vi "Test Data Dictionary API.vi"(8 "error in (no error)":errorcluster) -> (0 "error out":errorcluster)   [LabVIEW 2019]
uses:
  <vilib>/addons/_JKI Toolkits/Caraya/classes/Test/Test.lvclass
  LV-Data/LV-Data.lvclass
  LV-Data/Typedefs/Dictionary--cluster.ctl
  <vilib>/addons/_JKI Toolkits/Caraya/classes/Assert/Assert Equal Value and Type_Variant.vi
  <vilib>/addons/_JKI Toolkits/Caraya/classes/Assert/Assert.lvclass
  <vilib>/addons/_JKI Toolkits/Caraya/classes/Assert/Assert Not Error.vi
  <vilib>/numeric/Random Number (Range) I64.vi
  <vilib>/addons/_JKI Toolkits/Caraya/classes/Assert/Assert Error.vi
  LV-Data/API/XY-Data to Dictionary (Multiple).vi
  <vilib>/addons/_JKI Toolkits/Caraya/classes/Assert/Assert True.vi
  23d4e9fe-76af-4850-a45f-cc3c43636315.vi
  e87061af-0e9d-4de5-82b0-76289080f700.vi
  4053e775-25cb-4fab-9d61-351c3e686d1c.vi
  a8829717-a93e-4f97-b07c-db7713c6d1ae.vi
  8a392996-710f-4540-91e5-b205ccce4721.vi
  762a9f32-66e4-4e95-983a-dc45b51801a0.vi
  5820b508-eaf6-40a5-971f-30b0e9a2b10e.vi
  c95faebc-65c2-4475-abf8-9dea7ac9bcab.vi
  19599af3-a2bf-4e75-96ae-3692d4015444.vi
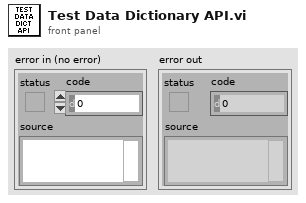
[diagram p1: front panel]
types:
  T1 = typedef "LV-Data.lvclass/Dictionary--cluster.ctl" = cluster{"key":string, "value":variant}
  T2 = typedef "LV-Data.lvclass/Map Variant--map.ctl" = map{string, variant}
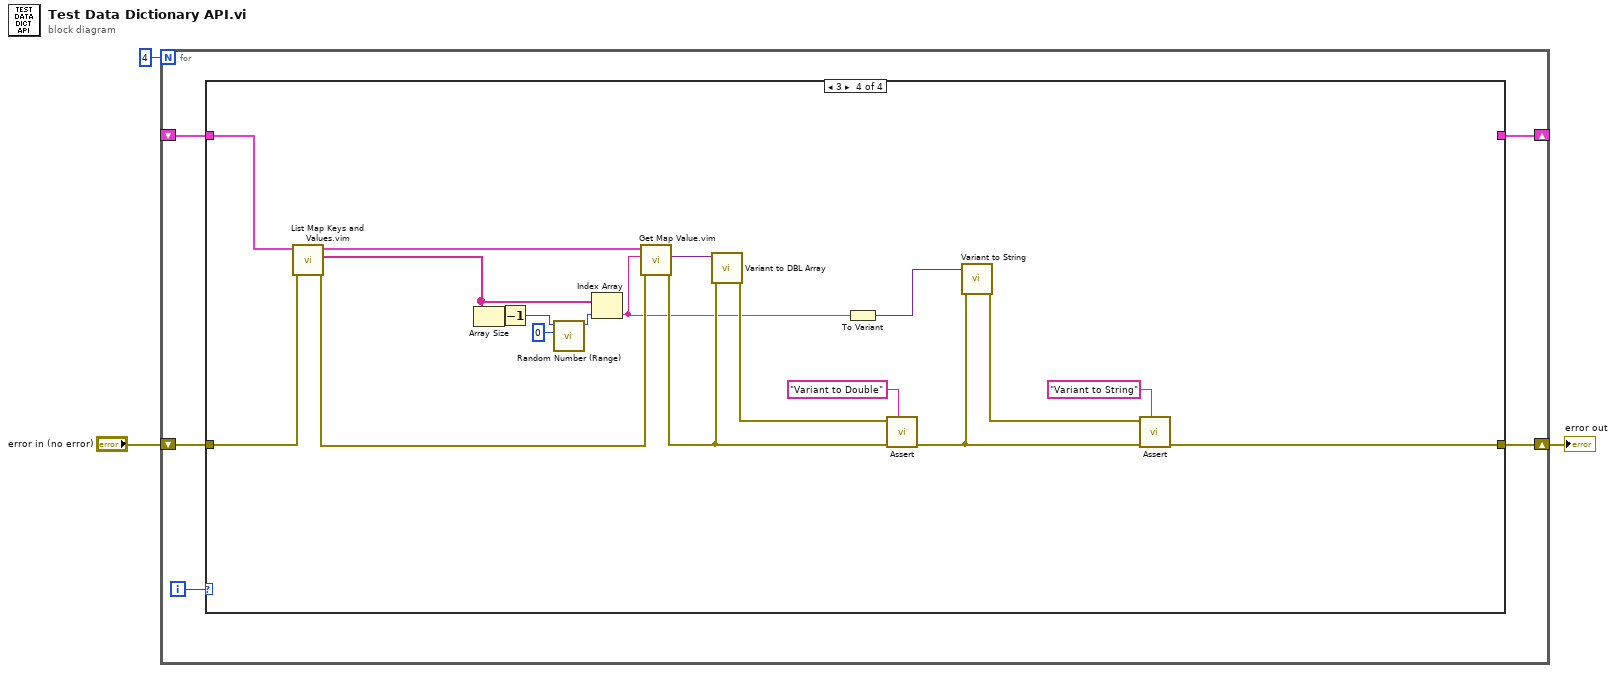
[diagram p0: block diagram]
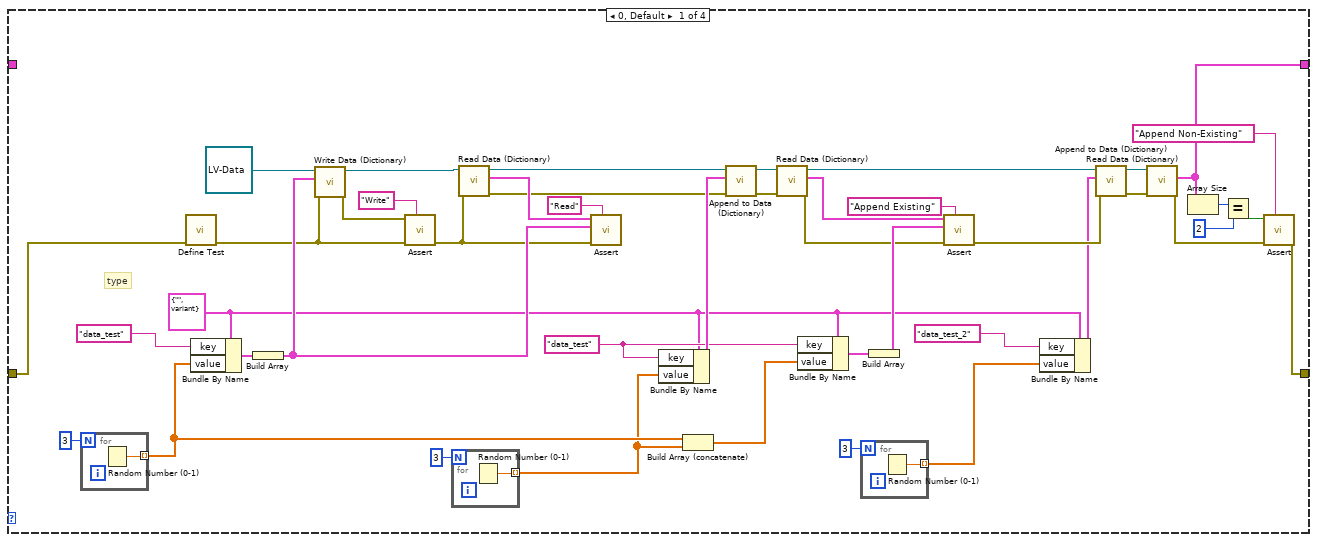
[diagram p2: hidden frame]
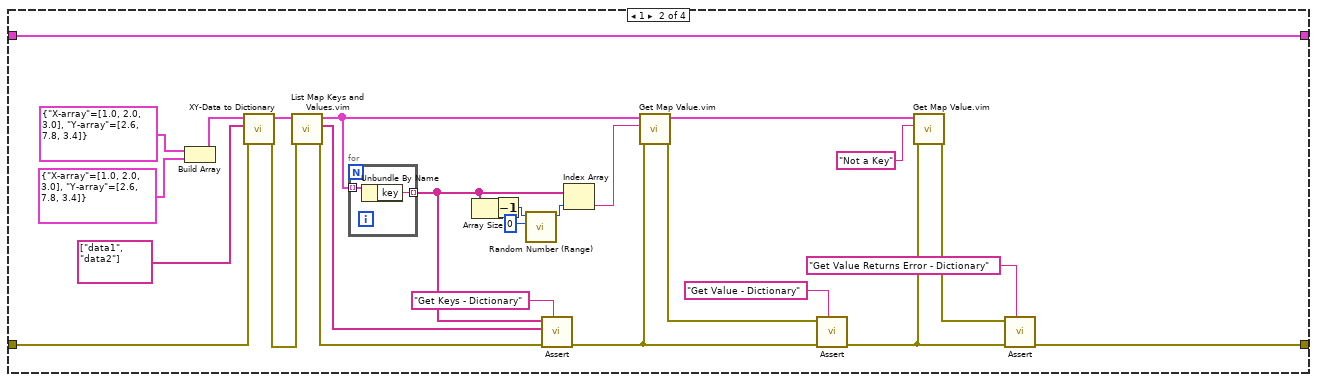
[diagram p3: hidden frame]
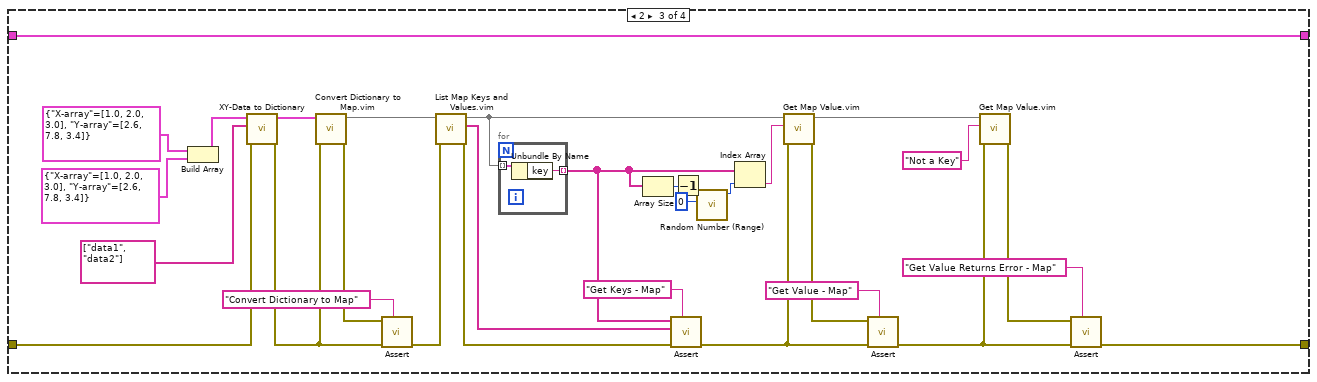
[diagram p4: hidden frame]
diagram:
  n1 = for {
    N: 4 -> [_]
    shift-right: [w7] -> w2
    shift-left: "error in (no error)" -> [w6]
    shift-right: [w5] -> _
    shift-left: _ -> [w4]
    i -> [w8]
    n2 = case shown="3" w8 {
      tunnel: [w17 w58 w87 w120] -> w7
      tunnel: w6 -> [w16 w60 w89 w130]
      tunnel: [w9 w56 w85 _] -> w5
      tunnel: w4 -> [_ w56 w85 w133]
      frame 0, Default {
        w43 = "data_test" ("key")
        w35 = T1 {"key"="", "value"=variant} ("key-value")
        # "type"
        n3 = for {
          N: 3 -> [_]
          tunnel: [w55] -> w14 mode=indexing
          n4 = Random Number (0-1)() -> (number: 0 to 1=w55:dbl)
        }
        n5 = call <vilib>:"Define Test.vi"("error in (no error)"=w16) -> ("error out"=w24:errorcluster)  [unwired: 10 in]
        n6 = Bundle By Name(cluster=w35, "key"="data_test", "value"=w14) -> (w51:T1)
        n7 = Build Array(w51) -> (w48:T1[])
        n8 = call "Write Data (Dictionary).vi"("error in (no error)"=w24, "Data (Dictionary)"=w48, "Data Save"=refnum<class "LV-Data.lvclass"> refnum) -> ("error out"=w25:errorcluster, "Data Save out"=w27:refnum<class "LV-Data.lvclass">)  [unwired: 7 in]
        n9 = call-poly <vilib>:"Assert.vi"("Label"="Write", "error in (no error)"=w24, "Not Error?"=w25) -> ("error out"=w26:errorcluster)  [unwired: 8 in]
        n10 = for {
          N: 3 -> [_]
          tunnel: [w54] -> w12 mode=indexing
          n11 = Random Number (0-1)() -> (number: 0 to 1=w54:dbl)
        }
        n12 = call "Read Data (Dictionary).vi"("error in (no error)"=w26, "Data Save"=w27) -> ("error out"=w23:errorcluster, "Data (Dictionary)"=w28:T1[], "Data Save out"=w22:refnum<class "LV-Data.lvclass">)  [unwired: 7 in]
        n13 = call-poly <vilib>:"Assert.vi"("Label"="Read", "error in (no error)"=w26, "Y"=w48, "X"=w28) -> ()  [unwired: 7 in, 1 out]
        n14 = Bundle By Name(cluster=w35, "key"=w43, "value"=w12) -> (w46:T1)
        n15 = Build Array (concatenate)(w14, w12) -> (w18:dbl[])
        n16 = call "Append to Data (Dictionary).vi"("error in (no error)"=w23, "key-value"=w46, "Data Save"=w22) -> ("error out"=w45:errorcluster, "Data Save out"=w44:refnum<class "LV-Data.lvclass">)  [unwired: 7 in]
        n17 = call "Read Data (Dictionary).vi"("error in (no error)"=w45, "Data Save"=w44) -> ("error out"=w21:errorcluster, "Data (Dictionary)"=w20:T1[], "Data Save out"=w19:refnum<class "LV-Data.lvclass">)  [unwired: 7 in]
        n18 = Bundle By Name(cluster=w35, "key"=w43, "value"=w18) -> (w42:T1)
        n19 = for {
          N: 3 -> [_]
          tunnel: [w53] -> w10 mode=indexing
          n20 = Random Number (0-1)() -> (number: 0 to 1=w53:dbl)
        }
        n21 = Build Array(w42) -> (w41:T1[])
        n22 = call-poly <vilib>:"Assert.vi"("Label"="Append Existing", "error in (no error)"=w21, "Y"=w41, "X"=w20) -> ("error out"=w37:errorcluster)  [unwired: 7 in]
        n23 = Bundle By Name(cluster=w35, "key"="data_test_2", "value"=w10) -> (w34:T1)
        n24 = call "Append to Data (Dictionary).vi"("error in (no error)"=w37, "key-value"=w34, "Data Save"=w19) -> ("error out"=w38:errorcluster, "Data Save out"=w39:refnum<class "LV-Data.lvclass">)  [unwired: 7 in]
        n25 = call "Read Data (Dictionary).vi"("error in (no error)"=w38, "Data Save"=w39) -> ("error out"=w30:errorcluster, "Data (Dictionary)"=w9:T1[])  [unwired: 7 in, 1 out]
        n26 = Array Size(array=w9) -> (size(s)=w33:i32)
        n27 = Equal?(x=w33, y=2) -> (x = y?=w31:bool)
        n28 = call-poly <vilib>:"Assert.vi"("Label"="Append Non-Existing", "error in (no error)"=w30, "True?"=w31) -> ("error out"=w17:errorcluster)  [unwired: 8 in]
      }
      frame 1 {
        n29 = Build Array(cluster{"X-array":dbl[], "Y-array":dbl[]} {"X-array"=[1.0, 2.0, 3.0], "Y-array"=[2.6, 7.8, 3.4]} ("XY-data in"), cluster{"X-array":dbl[], "Y-array":dbl[]} {"X-array"=[1.0, 2.0, 3.0], "Y-array"=[2.6, 7.8, 3.4]} ("XY-data in")) -> (w69:cluster{"X-array":dbl[], "Y-array":dbl[]}[])
        n30 = call-poly "XY-Data to Dictionary.vi"("error in (no error)"=w60, "Names"=string[] ["data1", "data2"], "XY-data in"=w69) -> ("error out"=w59:errorcluster, "Data (Dictionary)"=w70:T1[])  [unwired: 7 in]
        n31 = call "List Map Keys and Values.vim"("error in (no error)"=w59, "map in"=w70) -> ("error out"=w72:errorcluster, "Keys"=w71:string[], "map out"=w73:T1[])  [unwired: 6 in, 1 out]
        n32 = for {
          tunnel: w73 -> [w84] mode=indexing
          tunnel: [w83] -> w76 mode=indexing
          n33 = Unbundle By Name(w84) -> ("key"=w83:string)
        }
        n34 = Array Size(array=w76) -> (size(s)=w74:i32)
        n35 = Decrement(x=w74) -> (x-1=w57:i32)
        n36 = call-poly <vilib>:"Random Number (Range).vi"("lower bound (-100)"=i64 0, "upper bound (100)"=w57) -> ("number"=w75:i64)  [unwired: 9 in]
        n37 = call-poly <vilib>:"Assert.vi"("Label"="Get Keys - Dictionary", "error in (no error)"=w72, "Y"=w71, "X"=w76) -> ("error out"=w79:errorcluster)  [unwired: 7 in]
        n38 = Index Array(array=w76, index=w75) -> (element=w77:string)
        n39 = call "Get Map Value.vim"("error in (no error)"=w79, "Key"=w77, "map in"=w73) -> ("error out"=w78:errorcluster, "map out"=w80:T1[])  [unwired: 6 in, 1 out]
        n40 = call-poly <vilib>:"Assert.vi"("Label"="Get Value - Dictionary", "error in (no error)"=w79, "Not Error?"=w78) -> ("error out"=w82:errorcluster)  [unwired: 8 in]
        n41 = call "Get Map Value.vim"("error in (no error)"=w82, "Key"="Not a Key", "map in"=w80) -> ("error out"=w81:errorcluster)  [unwired: 6 in, 2 out]
        n42 = call-poly <vilib>:"Assert.vi"("Label"="Get Value Returns Error - Dictionary", "error in (no error)"=w82, "Error?"=w81) -> ("error out"=w58:errorcluster)  [unwired: 8 in]
      }
      frame 2 {
        n43 = Build Array(cluster{"X-array":dbl[], "Y-array":dbl[]} {"X-array"=[1.0, 2.0, 3.0], "Y-array"=[2.6, 7.8, 3.4]} ("XY-data in"), cluster{"X-array":dbl[], "Y-array":dbl[]} {"X-array"=[1.0, 2.0, 3.0], "Y-array"=[2.6, 7.8, 3.4]} ("XY-data in")) -> (w94:cluster{"X-array":dbl[], "Y-array":dbl[]}[])
        n44 = call-poly "XY-Data to Dictionary.vi"("error in (no error)"=w89, "Names"=string[] ["data1", "data2"], "XY-data in"=w94) -> ("error out"=w88:errorcluster, "Data (Dictionary)"=w90:T1[])  [unwired: 7 in]
        n45 = call "Convert Dictionary to Map.vim"("error in (no error)"=w88, "Data (Dictionary)"=w90) -> ("error out"=w101:errorcluster, "map out"=w104:T2)  [unwired: 8 in]
        n46 = call-poly <vilib>:"Assert.vi"("Label"="Convert Dictionary to Map", "error in (no error)"=w88, "Not Error?"=w101) -> ("error out"=w102:errorcluster)  [unwired: 8 in]
        n47 = call "List Map Keys and Values.vim"("error in (no error)"=w102, "map in"=w104) -> ("error out"=w103:errorcluster, "Keys"=w105:string[], "map out"=w109:T2)  [unwired: 6 in, 1 out]
        n48 = for {
          tunnel: w109 -> [w117] mode=indexing
          tunnel: [w116] -> w107 mode=indexing
          n49 = Unbundle By Name(w117) -> ("key"=w116:string)
        }
        n50 = Array Size(array=w107) -> (size(s)=w106:i32)
        n51 = call-poly <vilib>:"Assert.vi"("Label"="Get Keys - Map", "error in (no error)"=w103, "Y"=w105, "X"=w107) -> ("error out"=w112:errorcluster)  [unwired: 7 in]
        n52 = Decrement(x=w106) -> (x-1=w86:i32)
        n53 = call-poly <vilib>:"Random Number (Range).vi"("lower bound (-100)"=i64 0, "upper bound (100)"=w86) -> ("number"=w108:i64)  [unwired: 9 in]
        n54 = Index Array(array=w107, index=w108) -> (element=w110:string)
        n55 = call "Get Map Value.vim"("error in (no error)"=w112, "Key"=w110, "map in"=w109) -> ("error out"=w111:errorcluster, "map out"=w113:T2)  [unwired: 6 in, 1 out]
        n56 = call-poly <vilib>:"Assert.vi"("Label"="Get Value - Map", "error in (no error)"=w112, "Not Error?"=w111) -> ("error out"=w115:errorcluster)  [unwired: 8 in]
        n57 = call "Get Map Value.vim"("error in (no error)"=w115, "Key"="Not a Key", "map in"=w113) -> ("error out"=w114:errorcluster)  [unwired: 6 in, 2 out]
        n58 = call-poly <vilib>:"Assert.vi"("Label"="Get Value Returns Error - Map", "error in (no error)"=w115, "Error?"=w114) -> ("error out"=w87:errorcluster)  [unwired: 8 in]
      }
      frame 3 {
        n59 = call "List Map Keys and Values.vim"("error in (no error)"=w130, "map in"=w133) -> ("error out"=w129:errorcluster, "Keys"=w131:string[], "map out"=w132:T1[])  [unwired: 6 in, 1 out]
        n60 = Array Size(array=w131) -> (size(s)=w135:i32)
        n61 = Decrement(x=w135) -> (x-1=w124:i32)
        n62 = call-poly <vilib>:"Random Number (Range).vi"("lower bound (-100)"=i64 0, "upper bound (100)"=w124) -> ("number"=w136:i64)  [unwired: 9 in]
        n63 = Index Array(array=w131, index=w136) -> (element=w119:string)
        n64 = call "Get Map Value.vim"("error in (no error)"=w129, "Key"=w119, "map in"=w132) -> ("error out"=w125:errorcluster, "value"=w128:variant)  [unwired: 6 in, 1 out]
        n65 = call "Variant to DBL Array.vi"("error in (no error)"=w125, "Data (Variant)"=w128) -> ("error out"=w126:errorcluster)  [unwired: 7 in, 2 out]
        n66 = To Variant(anything=w119) -> (Variant=w118:variant)
        n67 = call-poly <vilib>:"Assert.vi"("Label"="Variant to Double", "error in (no error)"=w125, "Not Error?"=w126) -> ("error out"=w122:errorcluster)  [unwired: 8 in]
        n68 = call "Variant to String.vi"("error in (no error)"=w122, "Data (Variant)"=w118) -> ("error out"=w121:errorcluster)  [unwired: 8 in, 1 out]
        n69 = call-poly <vilib>:"Assert.vi"("Label"="Variant to String", "error in (no error)"=w122, "Not Error?"=w121) -> ("error out"=w120:errorcluster)  [unwired: 8 in]
      }
    }
  }
  "error out" <- w2
